vi "Choix type arret.vi"(0 "reg":string) -> (2 "Choix consigne locale : 2":T1 items=["Consignes actuelles", "Mesures actuelles", "Valeur fixe pour tous les régulateurs"], 3 "Valeur":dbl, 4 "annulé ?":bool)   [LabVIEW 2022 SP3]
uses:
  Enum/Commande Choix arret reg.ctl
panel:
  in  "annuler":bool
  in  "Bouton OK":bool
  in  "Valeur consigne locale (°C)":dbl=20.0
  in  "Choix consigne locale :":T1 items=["Consignes actuelles", "Mesures actuelles", "Valeur fixe pour tous les régulateurs"]
  # "ARRÊT DE LA RÉGULATION\npour les régulateurs :"
  # "Après arrêt du RUN, la consigne active sera la consigne locale.\n\nQuelle valeur souhaitez-vous donner à cette consigne locale :"
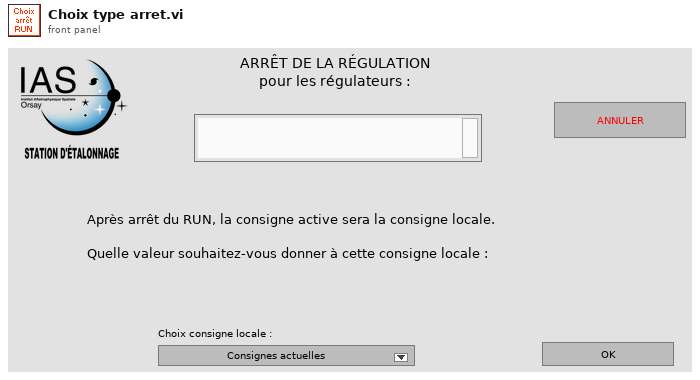
[diagram p1: front panel]
types:
  T1 = typedef "Commande Choix arret reg.ctl" = u16
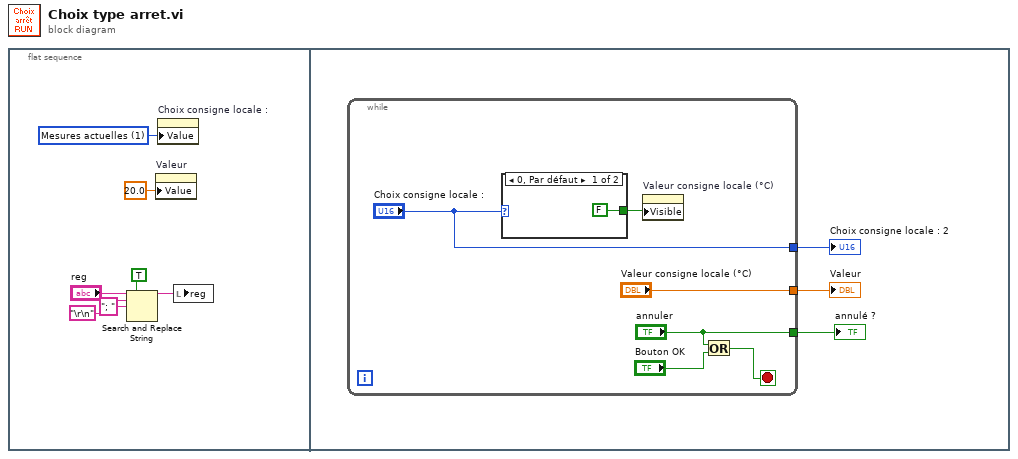
[diagram p0: block diagram]
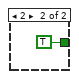
[diagram p2: hidden frame]
diagram:
  n1 = flat-sequence {
    frame #0 {
      w7 = T1 1 items=["Consignes actuelles", "Mesures actuelles", "Valeur fixe pour tous les régulateurs"] ("Choix consigne locale :")
      n2 = Search and Replace String(replace all?=TRUE ("tout remplacer ? (F)"), input string="reg", search string="\r\n", replace string="; " ("chaîne de remplacement (\"\")")) -> (result string=w1:string)  [unwired: 4 in, 3 out]
      n3 = property on="Valeur" class="NumNb (strict)"("Value"=20.0 ("Valeur")) -> ()  [unwired: 2 in, 2 out]
      n4 = property on="Choix consigne locale :" class="MDér (strict)"("Value"=w7) -> ()  [unwired: 2 in, 2 out]
      n5 = local write "reg"(w1) -> ()
    }
    frame #1 {
      n6 = while {
        tunnel: ["annuler"] -> w10
        tunnel: ["Choix consigne locale :"] -> w9
        tunnel: ["Valeur consigne locale (°C)"] -> w8
        stop <- w15 stop-if-true
        n7 = case shown="0, Par défaut" "Choix consigne locale :" {
          tunnel: [FALSE TRUE] -> w13
          frame 0, Default {
          }
          frame 2 {
          }
        }
        n8 = property on="Valeur consigne locale (°C)" class="NumNb (strict)"("Visible"=w13) -> ()  [unwired: 2 in, 2 out]
        n9 = Or(x="annuler", y="Bouton OK") -> (x .or. y?=w15:bool)
      }
      "annulé ?" <- w10
      "Choix consigne locale : 2" <- w9
      "Valeur" <- w8
    }
  }
